vi "Send RX Message.vi"(8 "error in (no error)":errorcluster, 10 "message":string, 11 "RxTx in":refnum<class "RxTx.lvclass">) -> (0 "error out":errorcluster, 3 "RxTx out":refnum<class "RxTx.lvclass">)   [LabVIEW 2018, in "RxTx.lvclass"]
uses:
  RxTx.lvclass
  RxTx.lvclass/RxTx.ctl
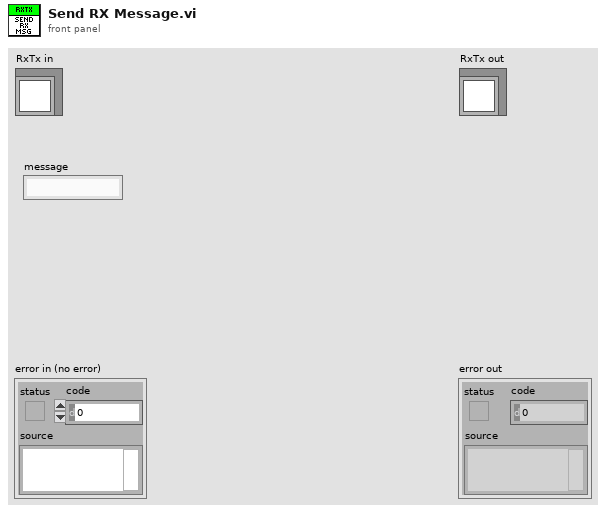
[diagram p1: front panel]
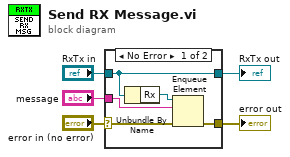
[diagram p0: block diagram]
diagram:
  n1 = case shown="No Error" "error in (no error)" {
    selector: "error in (no error)" -> [w9 w12]
    tunnel: [w10 w12] -> w3
    tunnel: [w7 w11] -> w2
    tunnel: "RxTx in" -> [w7 w11]
    tunnel: "message" -> [w6 _]
    frame No Error {
      n2 = Unbundle By Name(w7) -> ("Rx"=w8:refnum<queue>)
      n3 = Enqueue Element(queue=w8, element=w6, error in (no error)=w9) -> (error out=w10:errorcluster)  [unwired: 1 in, 2 out]
    }
    frame Error {
    }
  }
  "error out" <- w3
  "RxTx out" <- w2
